vi "get TurnTable Parameter.vi"(8 "error in (no error)":errorcluster caption="에러 입력(에러 없음)", 11 "CO3000 입력":refnum<class "CO3000.lvclass">) -> (0 "error out":errorcluster caption="에러 출력", 2 "Turn Table Info":T1 {"Target Angle" min=0.0 max=360.0}, 3 "CO3000 출력":refnum<class "CO3000.lvclass">)   [LabVIEW 2023, in "Turn Table and Mast.lvlib" / "CO3000.lvclass"]
uses:
  CO3000.lvclass
  CO3000.lvclass/CO3000.ctl
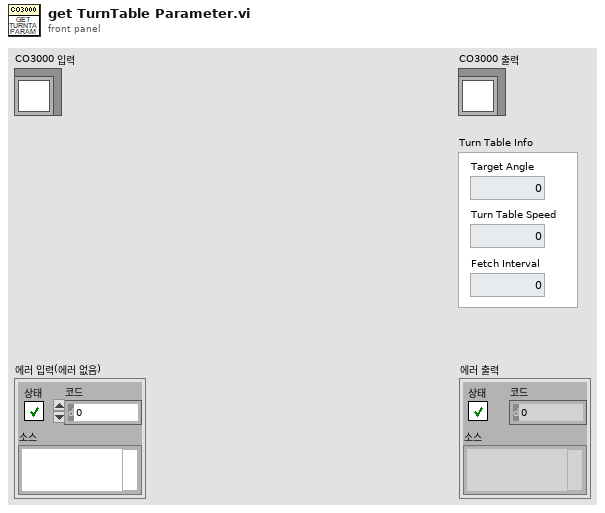
[diagram p1: front panel]
types:
  T1 = cluster{"Target Angle":dbl, "Turn Table Speed":i32, "Fetch Interval":i32}
  T2 = cluster{"Target Angle":dbl, "Speed":i32, "Fetch Interval":i32}
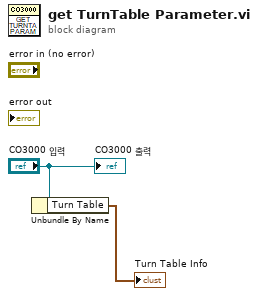
[diagram p0: block diagram]
diagram:
  n1 = Unbundle By Name("CO3000 입력") -> ("Turn Table"=→"Turn Table Info":T2)
  "CO3000 출력" <- "CO3000 입력"
